vi "Ecrire config REG.vi"(2 "error in (no error) 2":errorcluster caption="entrée d'erreur (pas d'erreur)", 3 "refnum 2":T1 caption="refnum") -> (0 "error out":errorcluster, 1 "refnum out":T1)   [LabVIEW 2022 SP3]
uses:
  <vilib>/Utility/config.llb/Config Data RefNum.ctl
  Variables globales/Variables glob EUROTHERM.vi
  <vilib>/Utility/config.llb/Write Key (String).vi
  <vilib>/Utility/config.llb/NI_LVConfig.lvlib
panel:
  out "COM":string[](array[string])
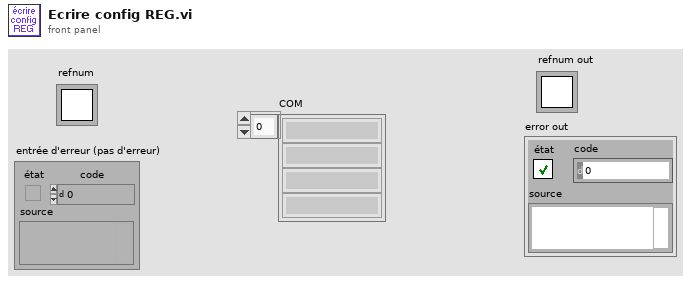
[diagram p1: front panel]
types:
  T1 = typedef "NI_LVConfig.lvlib/Config Data RefNum.ctl" = refnum<k1>
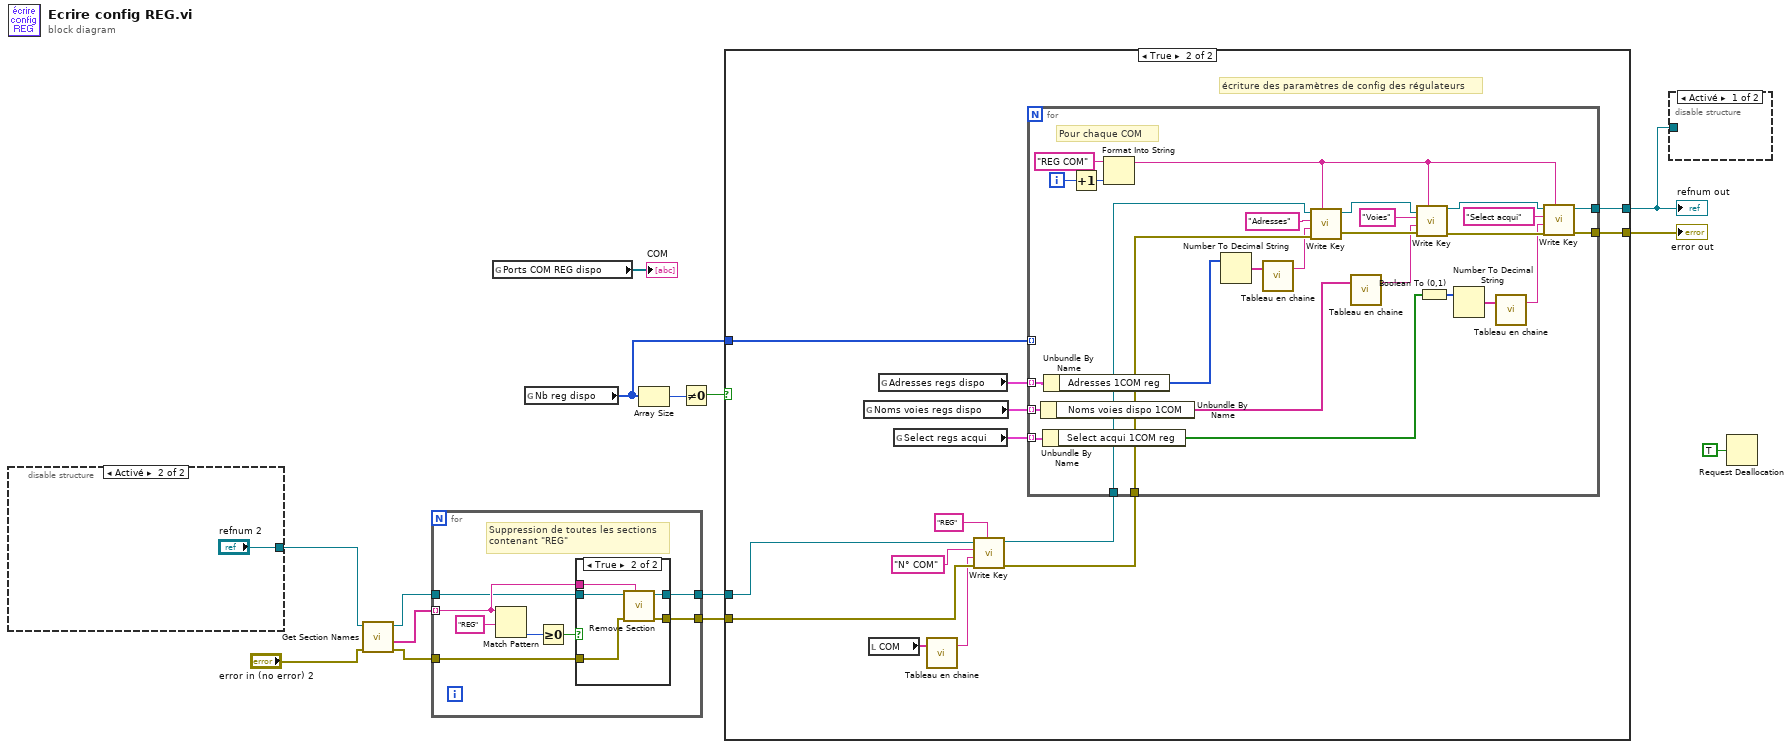
[diagram p0: block diagram]
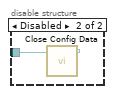
[diagram p2: hidden frame]
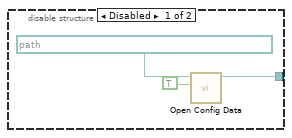
[diagram p3: hidden frame]
diagram:
  n1 = disable-structure shown="Activé" {
    disable-tunnel: [w15 "refnum 2"] -> w3
    frame Disabled {
      n2 = call <vilib>:"Open Config Data.vi"("create file if necessary (T)"=TRUE ("create file if necessary? (T)"), "configuration file path"=path "C:/LABVIEW/PRES+TEMP+REG dernière version/Configurations/config acqui.ini") -> ("refnum"=w15:T1)  [unwired: 7 in, 2 out]
    }
    frame Enabled {
    }
  }
  n3 = call <vilib>:"Get Section Names.vi"("error in (no error)"="error in (no error) 2", "refnum"=w3) -> ("error out"=w7:errorcluster, "section names"=w5:string[], "refnum out"=w6:T1)  [unwired: 7 in]
  n4 = for {
    tunnel: w5 -> [w23] mode=indexing
    tunnel: w6 -> [w22]
    tunnel: w7 -> [w21]
    tunnel: [w20] -> w9
    tunnel: [w19] -> w10
    # "Suppression de toutes les sections\ncontenant \"REG\""
    n5 = Match Pattern(string=w23, regular expression="REG" ("expression régulière")) -> (offset past match=w25:i32)  [unwired: 1 in, 3 out]
    n6 = Greater Or Equal To 0?(x=w25) -> (x >= 0?=w24:bool)
    n7 = case shown="True" w24 {
      tunnel: w23 -> [_ w33]
      tunnel: w22 -> [w28 w32]
      tunnel: w21 -> [w27 w31]
      tunnel: [w28 w30] -> w20
      tunnel: [w27 w29] -> w19
      frame False {
      }
      frame True {
        n8 = call <vilib>:"Remove Section.vi"("section"=w33, "error in (no error)"=w31, "refnum"=w32) -> ("error out"=w29:errorcluster, "refnum out"=w30:T1)  [unwired: 6 in, 1 out]
      }
    }
  }
  n9 = global read "Variables glob EUROTHERM.vi" "Ports COM REG dispo"() -> (→"COM":refnum<visa-resource-name>[])
  n10 = global read "Variables glob EUROTHERM.vi" "Nb reg dispo"() -> (w1:u8[])
  n11 = Array Size(array=w1) -> (size(s)=w11:i32)
  n12 = Not Equal To 0?(x=w11) -> (x != 0?=w12:bool)
  n13 = case shown="True" w12 {
    tunnel: w9 -> [w35 w49]
    tunnel: w10 -> [w34 w48]
    tunnel: [w35 w46] -> w2
    tunnel: [w34 w45] -> w13
    tunnel: w1 -> [_ w44]
    frame False {
    }
    frame True {
      # "écriture des paramètres de config des régulateurs"
      n14 = global read "Variables glob EUROTHERM.vi" "Noms voies regs dispo"() -> (w42:cluster{"Noms voies dispo 1COM":string[]}[])
      n15 = local read "COM"() -> (w39:string[])
      n16 = global read "Variables glob EUROTHERM.vi" "Adresses regs dispo"() -> (w43:cluster{"Adresses 1COM reg":u16[]}[])
      n17 = global read "Variables glob EUROTHERM.vi" "Select regs acqui"() -> (w41:cluster{"Select acqui 1COM reg":bool[]}[])
      n18 = call "Tableau en chaine.vi"("Tableau 1D"=w39) -> ("Chaîne"=w38:string)  [unwired: 1 in, 1 out]
      n19 = call-poly <vilib>:"Write Key.vi"("section"="REG", "error in (no error)"=w48, "value"=w38, "key"="N° COM", "refnum"=w49) -> ("error out"=w36:errorcluster, "refnum out"=w37:T1)  [unwired: 4 in, 1 out]
      n20 = for {
        tunnel: w37 -> [w71]
        tunnel: w36 -> [w70]
        tunnel: [w57] -> w46
        tunnel: [w56] -> w45
        tunnel: w44 -> [_] mode=indexing
        tunnel: w43 -> [w63] mode=indexing
        tunnel: w42 -> [w61] mode=indexing
        tunnel: w41 -> [w60] mode=indexing
        i -> [w65]
        # "Pour chaque COM"
        n21 = Unbundle By Name(w61) -> ("Noms voies dispo 1COM"=w53:string[])
        n22 = Unbundle By Name(w60) -> ("Select acqui 1COM reg"=w59:bool[])
        n23 = Unbundle By Name(w63) -> ("Adresses 1COM reg"=w62:u16[])
        n24 = Increment(x=w65) -> (x+1=w76:i32)
        n25 = Format Into String(initial string="REG COM" ("chaîne initiale"), w76) -> (resulting string=w64:string)  [unwired: 2 in, 1 out]
        n26 = Number To Decimal String(number=w62) -> (decimal integer string=w55:string[])  [unwired: 1 in]
        n27 = call "Tableau en chaine.vi"("Tableau 1D"=w55) -> ("Chaîne"=w54:string)  [unwired: 1 in, 1 out]
        n28 = call-poly <vilib>:"Write Key.vi"("section"=w64, "error in (no error)"=w70, "value"=w54, "key"="Adresses", "refnum"=w71) -> ("error out"=w68:errorcluster, "refnum out"=w69:T1)  [unwired: 4 in, 1 out]
        n29 = call "Tableau en chaine.vi"("Tableau 1D"=w53) -> ("Chaîne"=w52:string)  [unwired: 1 in, 1 out]
        n30 = call-poly <vilib>:"Write Key.vi"("section"=w64, "error in (no error)"=w68, "value"=w52, "key"="Voies", "refnum"=w69) -> ("error out"=w66:errorcluster, "refnum out"=w67:T1)  [unwired: 4 in, 1 out]
        n31 = Boolean To (0,1)(Boolean=w59) -> (0, 1=w58:i16[])
        n32 = Number To Decimal String(number=w58) -> (decimal integer string=w51:string[])  [unwired: 1 in]
        n33 = call "Tableau en chaine.vi"("Tableau 1D"=w51) -> ("Chaîne"=w50:string)  [unwired: 1 in, 1 out]
        n34 = call-poly <vilib>:"Write Key.vi"("section"=w64, "error in (no error)"=w66, "value"=w50, "key"="Select acqui", "refnum"=w67) -> ("error out"=w56:errorcluster, "refnum out"=w57:T1)  [unwired: 4 in, 1 out]
      }
    }
  }
  "refnum out" <- w2
  "error out" <- w13
  n35 = disable-structure shown="Activé" {
    disable-tunnel: w2 -> [_ w77]
    frame Enabled {
    }
    frame Disabled {
      n36 = call <vilib>:"Close Config Data.vi"("refnum"=w77) -> ()  [unwired: 9 in, 2 out]
    }
  }
  n37 = Request Deallocation(TRUE ("flag")) -> ()
